vi "filter possible timestamps stored as strings.vi"(11 "possible timestamps":T1(array[cluster])) -> (2 "property-to-match -> timestamp and original prop":T3(c390), 3 "remaining properties":T2(array[cluster]))   [LabVIEW 2020, in "nominal teststand model sequence support.lvlib"]
uses:
  nominal teststand model sequence support.lvlib
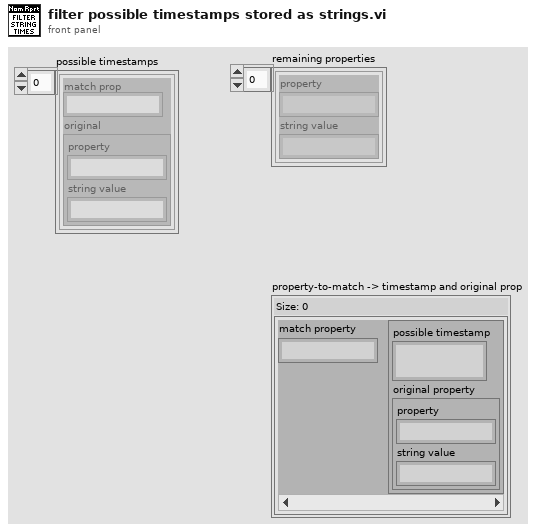
[diagram p1: front panel]
types:
  T1 = cluster{"match prop":string, "original":cluster{"property":string, "string value":string}}[]
  T2 = cluster{"property":string, "string value":string}[]
  T3 = map{string, cluster{"possible timestamp":timestamp, "original property":cluster{"property":string, "string value":string}}}
  T4 = cluster{"property":string, "string value":string}
  T5 = cluster{"time":timestamp, "original":cluster{"property":string, "string value":string}}
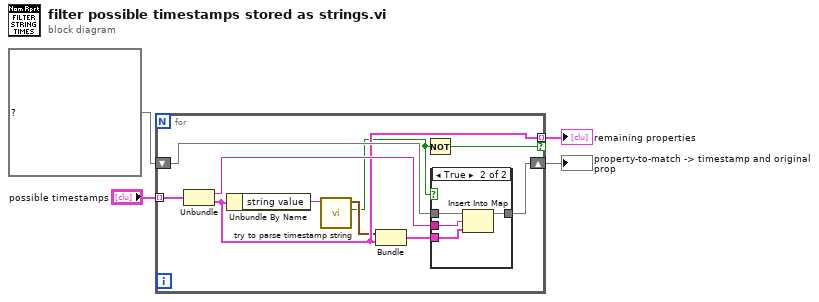
[diagram p0: block diagram]
diagram:
  n1 = for {
    tunnel: "possible timestamps" -> [w14] mode=indexing
    tunnel: [w10] -> w3 mode=indexing if=w6
    shift-right: [w13] -> w4
    shift-left: T3 {} ("property-to-match -> timestamp and original prop") -> [w12]
    n2 = Unbundle(w14) -> ("match prop"=w11:string, "original"=w10:T4)
    n3 = Unbundle By Name(w10) -> ("string value"=w8:string)
    n4 = call "try to parse timestamp string.vi"("possible timestamp string"=w8) -> ("valid"=w5:bool, "time"=w7:timestamp)  [unwired: 9 in]
    n5 = Bundle("time"=w7, "original"=w10) -> (w9:T5)  [unwired: 1 in]
    n6 = Not(x=w5) -> (.not. x?=w6:bool)
    n7 = case shown="True" w5 {
      tunnel: [w15 w19] -> w13
      tunnel: w12 -> [w15 w18]
      tunnel: w11 -> [_ w17]
      tunnel: w9 -> [_ w16]
      frame False {
      }
      frame True {
        n8 = Insert Into Map(map in=w18, key=w17, value=w16) -> (map out=w19:T3)  [unwired: 2 out]
      }
    }
  }
  "property-to-match -> timestamp and original prop" <- w4
  "remaining properties" <- w3
